vi "Scale List Add Item.vi"(9 "Sacle Setting Out":T1, 10 "r坐标轴列表":refnum<vi>, 11 "Data Viewer in":refnum<class "Data Viewer.lvclass">) -> (3 "Data Viewer out":refnum<class "Data Viewer.lvclass">)   [LabVIEW 2020, in "Data Viewer.lvlib" / "Data Viewer.lvclass"]
uses:
  Data Viewer.lvclass
  Scale Setting--cluster.ctl
  Data Viewer.lvclass/Data Viewer.ctl
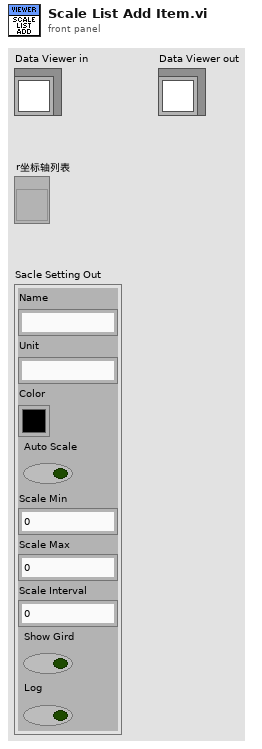
[diagram p1: front panel]
types:
  T1 = typedef "Data Viewer.lvlib/Data Viewer.lvclass/Scale Setting--cluster.ctl" = cluster{"Name":string, "Unit":string, "Color":u32, "Auto Scale":bool, "Scale Min":dbl, "Scale Max":dbl, "Scale Interval":dbl, "Show Gird":bool, "Log":bool}
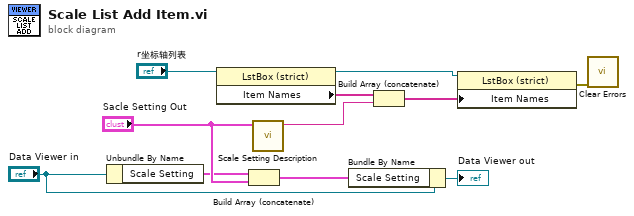
[diagram p0: block diagram]
diagram:
  n1 = Unbundle By Name("Data Viewer in") -> ("Scale Setting"=w1:T1[])
  n2 = property class="LstBox (strict)"(reference="r坐标轴列表") -> (reference out=w10:refnum<vi>, "Item Names"=w6:string[])  [unwired: 1 in, 1 out]
  n3 = Build Array (concatenate)(w1, "Sacle Setting Out") -> (w4:T1[])
  n4 = call "Scale Setting Description.vi"("Sacle Setting Out"="Sacle Setting Out") -> ("Description"=w9:string)  [unwired: 10 in]
  n5 = Bundle By Name(cluster="Data Viewer in", "Scale Setting"=w4) -> (→"Data Viewer out":refnum<class "Data Viewer.lvclass">)
  n6 = Build Array (concatenate)(w6, w9) -> (w7:string[])
  n7 = property class="LstBox (strict)"(reference=w10, "Item Names"=w7) -> (error out=w11:errorcluster)  [unwired: 1 in, 1 out]
  n8 = call <vilib>:"Clear Errors.vi"("error in (no error)"=w11) -> ()  [unwired: 5 in, 2 out]
